vi "gmap_example_PXI5671.vi"() -> ()   [LabVIEW 2025]
uses:
  <vilib>/sklein/WebView2 XControl/WebView2 XControl/WebView2 Control.xctl
panel:
  out "Map file":string="file:///C:/Users/Slava/Documents/DATA/WORK/Projects/GMAPSv2/123.html"
  in  "Route altitude, feet":dbl
  in  "Route speed, mph":dbl
  out "Trackfile Generation":u8(slide) scale=0.0..100.0
  out "GNSS signal generation started?":bool
  out "Trackfile generation in progress":bool
  out "Coordinates":string
  in  "Send route":bool
  out "WebView2 Browser Control":string(xcontrol)
  in  "Refresh map":bool
  out "Status":string
  in  "stop":bool
  # "GNSS Simulation System (GPS Constellation)"
  # "Route options"
  # "System status"
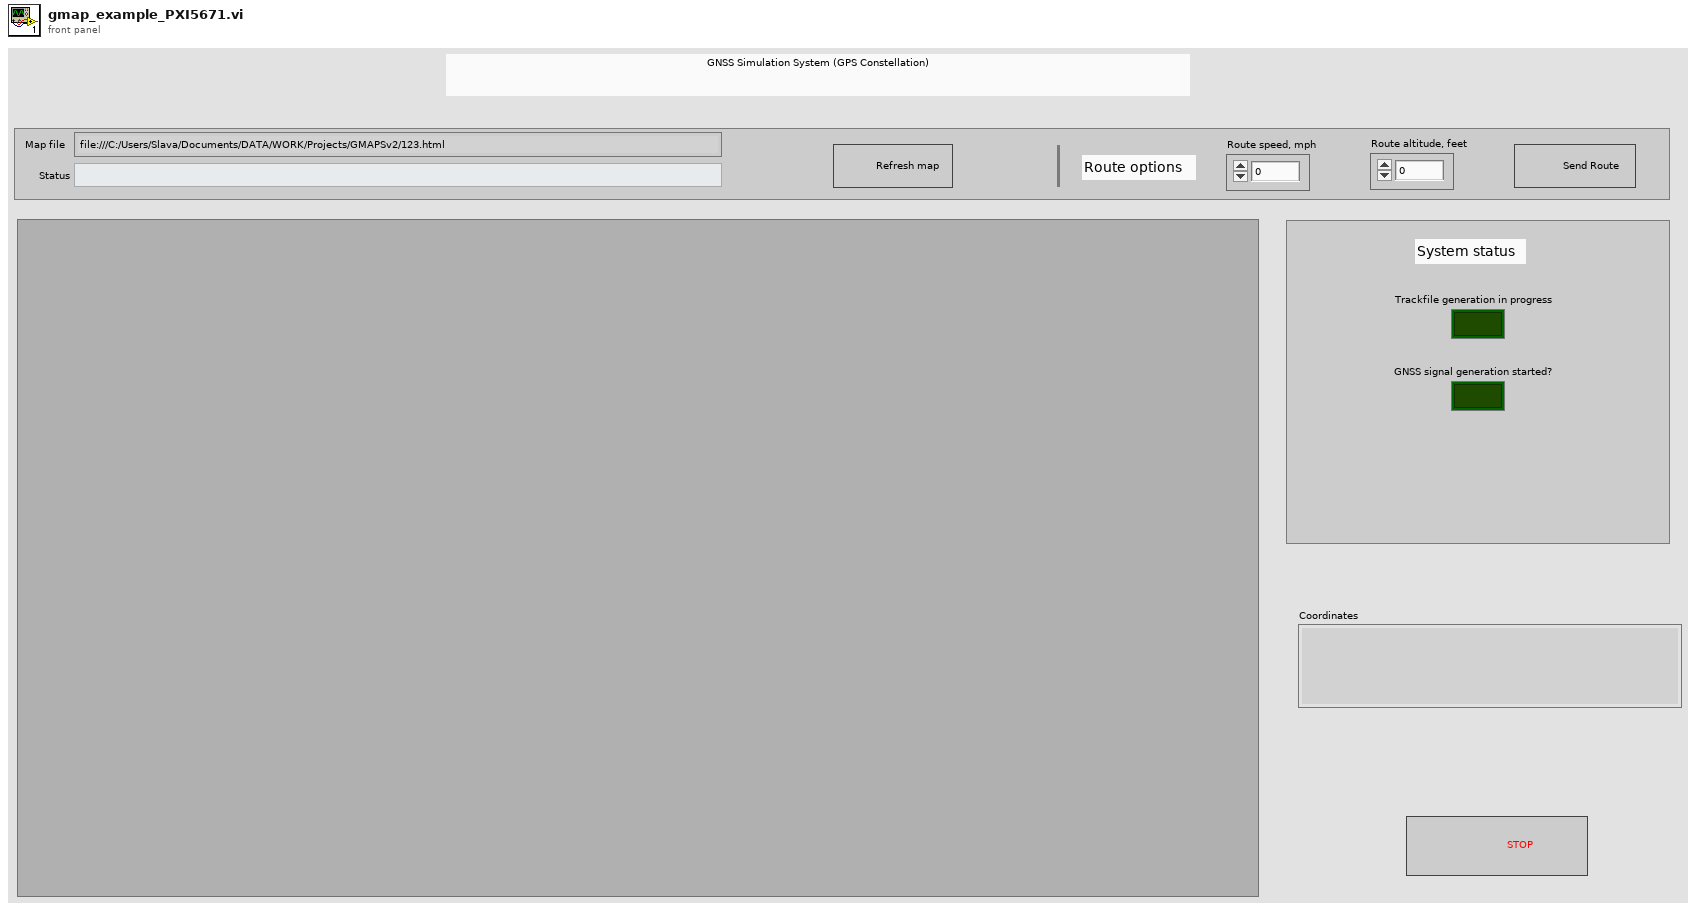
[diagram p1: front panel]
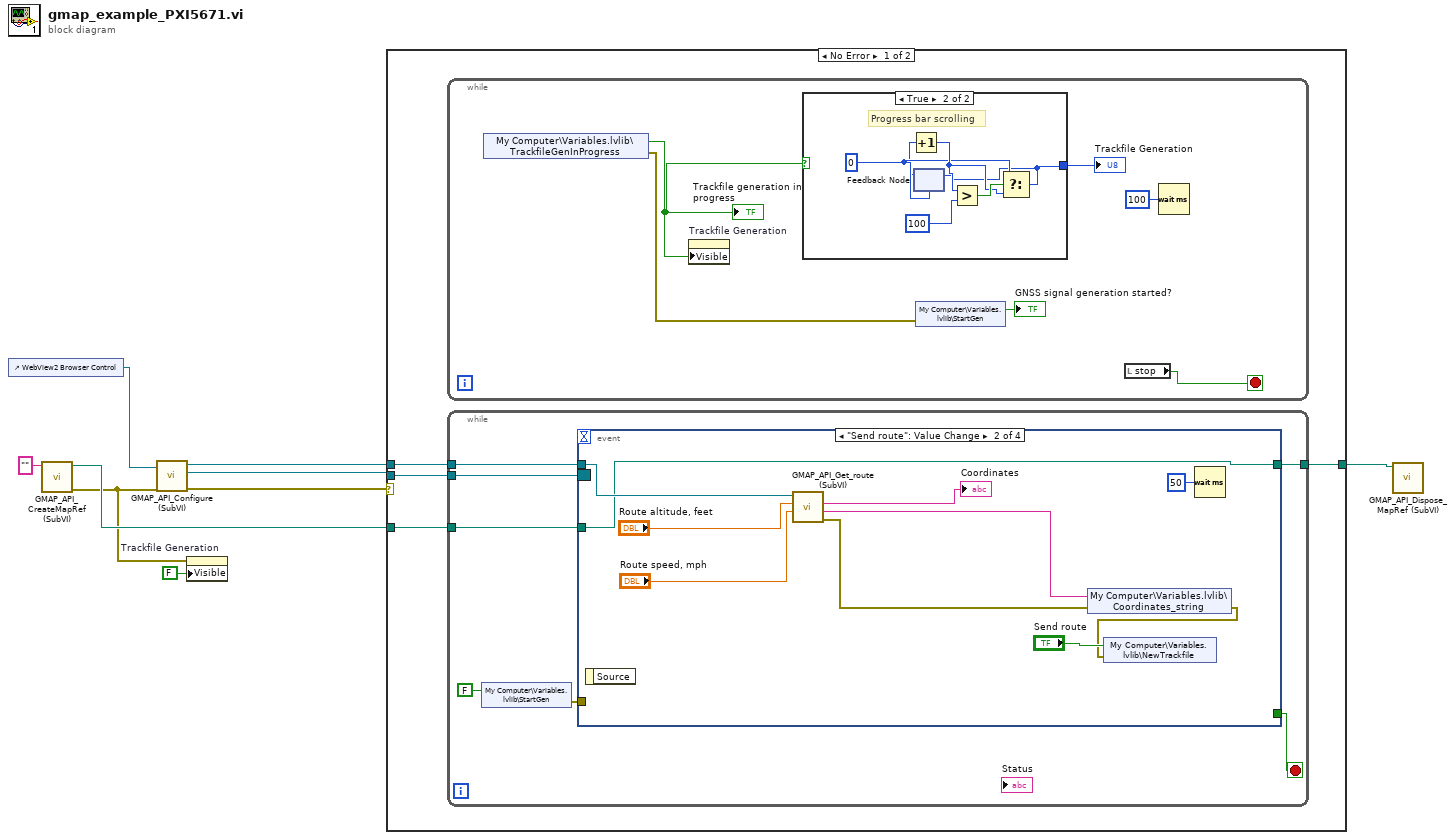
[diagram p0: block diagram]
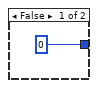
[diagram p2: hidden frame]
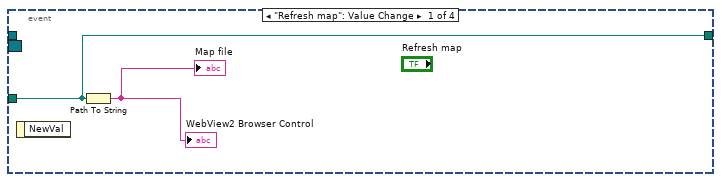
[diagram p3: hidden frame]
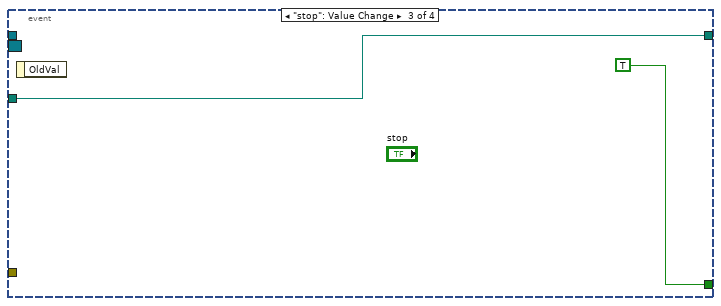
[diagram p4: hidden frame]
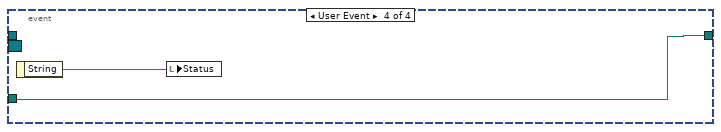
[diagram p5: hidden frame]
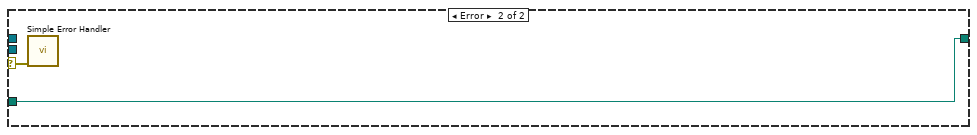
[diagram p6: hidden frame]
diagram:
  n1 = control-ref of="WebView2 Browser Control"() -> (w5:refnum<vi>)
  n2 = call "GMAP_API_CreateMapRef (SubVI).vi"("Gmaps API key"="") -> ("error out"=w2:errorcluster, "map file path"=w3:path)  [unwired: 9 in]
  n3 = call "GMAP_API_Configure (SubVI).vi"("error in"=w2, "Browser control in"=w5) -> ("error out"=w8:errorcluster, "Event Registration Refnum"=w9:refnum<event-registration>, "Browser control out"=w7:refnum<vi>)  [unwired: 7 in]
  n4 = property on="Trackfile Generation" class="Slide (strict)"(error in=w2, "Visible"=FALSE) -> ()  [unwired: 1 in, 2 out]
  n5 = case shown="No Error" w8 {
    selector: w8 -> [_ w51]
    tunnel: w9 -> [w13 _]
    tunnel: w7 -> [w12 _]
    tunnel: w3 -> [w11 w50]
    tunnel: [w10 w50] -> w1
    frame No Error {
      n6 = while {
        stop <- w19 stop-if-true
        n7 = shared-variable "My Computer\\Variables.lvlib\\TrackfileGenInProgress"() -> (w15:bool, error out=w14:errorcluster)  [unwired: 1 in]
        "Trackfile generation in progress" <- w15
        n8 = property on="Trackfile Generation" class="Slide (strict)"("Visible"=w15) -> ()  [unwired: 2 in, 2 out]
        n9 = case shown="True" w15 {
          tunnel: [0 w21] -> w16
          frame False {
          }
          frame True {
            w23 = 0
            # "Progress bar scrolling"
            n10 = feedback #1(w23) -> (w22:i32)
            n11 = Increment(x=w22) -> (x+1=w24:i32)
            n12 = Greater?(x=w24, y=100) -> (0:w25:bool)
            n13 = Select(t=w23, s=w25, f=w24) -> (s? t:f=w21:i32)
            n14 = feedback-in #1(w21) -> ()
          }
        }
        "Trackfile Generation" <- w16
        n15 = shared-variable "My Computer\\Variables.lvlib\\StartGen"(error in=w14) -> (→"GNSS signal generation started?":bool)  [unwired: 1 out]
        n16 = local read "stop"() -> (w19:bool)
        n17 = Wait (ms)(milliseconds to wait=u32 100) -> ()  [unwired: 1 out]
      }
      n18 = while {
        tunnel: w13 -> [w33]
        tunnel: w12 -> [w31]
        tunnel: w11 -> [w28]
        tunnel: [w27] -> w10
        stop <- w32 stop-if-true
        n19 = shared-variable "My Computer\\Variables.lvlib\\StartGen"(FALSE ("StartGen")) -> (error out=w30:errorcluster)  [unwired: 1 in]
        n20 = event shown="[1] \"Send route\": Value Change" {
          selector: w33 -> [_ _ _ _]
          dyn-events: _ -> [_ _ _ _]
          timeout: _ -> [_ _ _ _]
          tunnel: [_ _ TRUE _] -> w32
          tunnel: w31 -> [_ w45 _ _]
          tunnel: w30 -> [_ _ _ _]
          tunnel: w28 -> [w35 w36 w46 w48]
          tunnel: [w35 w36 w46 w48] -> w27
          event "Refresh map": Value Change {
            n21 = event-data() -> ()  [unwired: 1 in, 1 out]
            n22 = Path To String(path=w35) -> (string=→"WebView2 Browser Control" →"Map file":string)
          }
          event "Send route": Value Change {
            n23 = event-data() -> ()  [unwired: 1 in, 1 out]
            n24 = call "GMAP_API_Get_route (SubVI).vi"("Route speed, mph"="Route speed, mph", "Route altitude, feet"="Route altitude, feet", "Browser control ref in"=w45) -> ("error out"=w41:errorcluster, "Coordinates string (out)"=w37:string, "Coordinates"=→"Coordinates":string)  [unwired: 5 in, 1 out]
            n25 = shared-variable "My Computer\\Variables.lvlib\\Coordinates_string"(w37, error in=w41) -> (error out=w42:errorcluster)
            n26 = shared-variable "My Computer\\Variables.lvlib\\NewTrackfile"("Send route", error in=w42) -> ()  [unwired: 1 out]
            n27 = Wait (ms)(milliseconds to wait=u32 50) -> ()  [unwired: 1 out]
          }
          event "stop": Value Change {
            n28 = event-data() -> ()  [unwired: 1 in, 1 out]
          }
          event User Event {
            n29 = event-data() -> ("String"=w49:string)  [unwired: 1 in]
            n30 = local write "Status"(w49) -> ()
          }
        }
      }
    }
    frame Error {
      n31 = call <vilib>:"Simple Error Handler.vi"("error in (no error)"=w51) -> ()  [unwired: 4 in, 5 out]
    }
  }
  n32 = call "GMAP_API_Dispose_MapRef (SubVI).vi"("map file path"=w1) -> ()  [unwired: 10 in, 1 out]
